vi "Strip Path.vi"   [LabVIEW 2020, in "openg_file.lvlib"]
doc: "Functions identically to LabVIEW \"Strip Path\" function, but is polymorphic to also allow the path input to be an array. If an array is used, the outputs become arrays."
uses:
  openg_file.lvlib
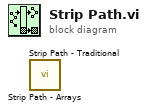
[diagram p0: block diagram]
diagram:
  n1 = call "Strip Path - Arrays.vi"() -> ()  [unwired: 1 in, 2 out]
  n2 = call "Strip Path - Traditional.vi"() -> ()  [unwired: 1 in, 2 out]
